vi "Get Window Width and Height.vi"(8 "error in":errorcluster, 11 "hWnd in":u32) -> (0 "error out":errorcluster, 1 "Width":i32, 2 "Height":i32, 3 "hWnd out":u32)   [LabVIEW 2019, in "Screenshot Utility.lvlib"]
uses:
  Screenshot Utility.lvlib
  User32.dll
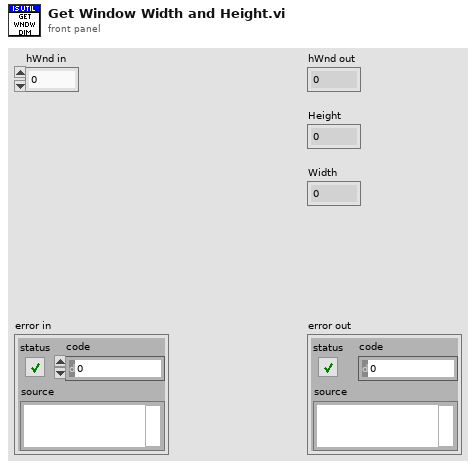
[diagram p1: front panel]
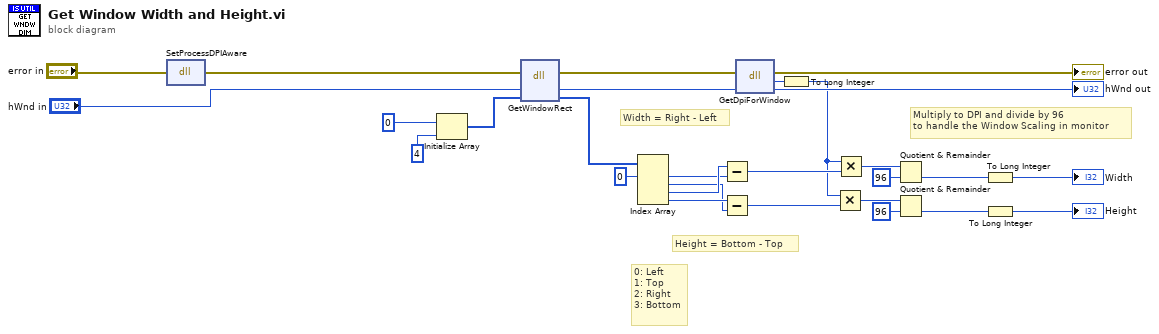
[diagram p0: block diagram]
diagram:
  # "Multiply to DPI and divide by 96\nto handle the Window Scaling in monitor"
  # "Height = Bottom - Top"
  # "Width = Right - Left"
  # "0: Left\n1: Top\n2: Right\n3: Bottom"
  n1 = dll-call lib="user32.dll" fn="SetProcessDPIAware"(error in="error in") -> (error out=w24:errorcluster)  [unwired: 2 in, 2 out]
  n2 = Initialize Array(0, 4 ("dimension size")) -> (w11:i32[])
  n3 = dll-call lib="user32.dll" fn="GetWindowRect"(error in=w24, "hWnd"="hWnd in", "lpRect"=w11) -> (error out=w16:errorcluster, "hWnd"=w18:u32, "lpRect"=w6:i32[])  [unwired: 2 in, 2 out]
  n4 = Index Array(array=w6, index #1=0 ("index")) -> (element #1=w9:i32, element #2=w8:i32, element #3=w14:i32, element #4=w15:i32)  [unwired: 3 in]
  n5 = Subtract(x=w14, y=w9) -> (x-y=w19:i32)
  n6 = Subtract(x=w15, y=w8) -> (x-y=w22:i32)
  n7 = dll-call lib="user32.dll" fn="GetDpiForWindow"(error in=w16, "hWnd"=w18) -> (error out=→"error out":errorcluster, "return"=w23:u32, "hWnd"=→"hWnd out":u32)  [unwired: 2 in, 1 out]
  n8 = To Long Integer(number=w23) -> (32bit integer=w5:i32)
  n9 = Multiply(x=w5, y=w22) -> (x*y=w1:i32)
  n10 = Multiply(x=w5, y=w19) -> (x*y=w2:i32)
  n11 = Quotient & Remainder(x=w2, y=96) -> (floor(x/y)=w20:i32)  [unwired: 1 out]
  n12 = Quotient & Remainder(x=w1, y=96) -> (floor(x/y)=w21:i32)  [unwired: 1 out]
  n13 = To Long Integer(number=w20) -> (32bit integer=→"Width":i32)
  n14 = To Long Integer(number=w21) -> (32bit integer=→"Height":i32)
